vi "Autobuild Main.vi"() -> ()   [LabVIEW 2022 SP3]
uses:
  subVIs/Package Builder API/build type.ctl
  subVIs/Package Builder API/NI Package Builder API.lvlib
panel:
  out "current build":i32
  out "total builds":i32
  in  "Build Package":bool=TRUE
  in  "Build EXEs":bool=TRUE
  in  "Tab Control":T1(tab)
  in  "Projects":path[](array[path])=[path "C:/dev/class-d-amplifier/source/crosstalk/Crosstalk_Class D Amplifier.lvproj", path "C:/dev/class-d-amplifier/source/single tone/Single Tone Measurements_Class D Amplifier.lvproj", path "C:/dev/class-d-amplifier/source/stepped frequency sweep/Stepped Frequency Sweep_Class D Amplifier.lvproj", path "C:/dev/class-d-amplifier/source/efficiency/Efficiency_Class D Amplifier.lvproj", path "C:/dev/class-d-amplifier/source/efficiency sweep/Efficiency Sweep_Class D Amplifier.lvproj", path "C:/dev/class-d-amplifier/source/generation/Generation_Class D Amplifier.lvproj", path "C:/dev/class-d-amplifier/source/single tone no gen/Single Tone No Gen_Class D Amplifier.lvproj", path "C:/dev/class-d-amplifier/source/single tone power sweep/Single Tone Power Sweep.lvproj", path "C:/dev/class-d-amplifier/source/noise sweep/Noise Sweep_Class D Amplifier.lvproj", path "C:/dev/class-d-amplifier/source/crosstalk sweep/Crosstalk Sweep.lvproj"]
  in  "background service":path=path "C:/dev/class-d-amplifier/source/service/generation/Audio Generation Service.lvproj"
  in  "utilities":path=path "C:/dev/class-d-amplifier/source/service/register service/RegisterServices.lvproj"
  out "command line standard output":string
  in  "package builder solution path":path=path "C:/dev/class-d-amplifier/package/ClassDAmplifier.pbs"
  in  "error in (no error)":errorcluster
  out "error out":errorcluster
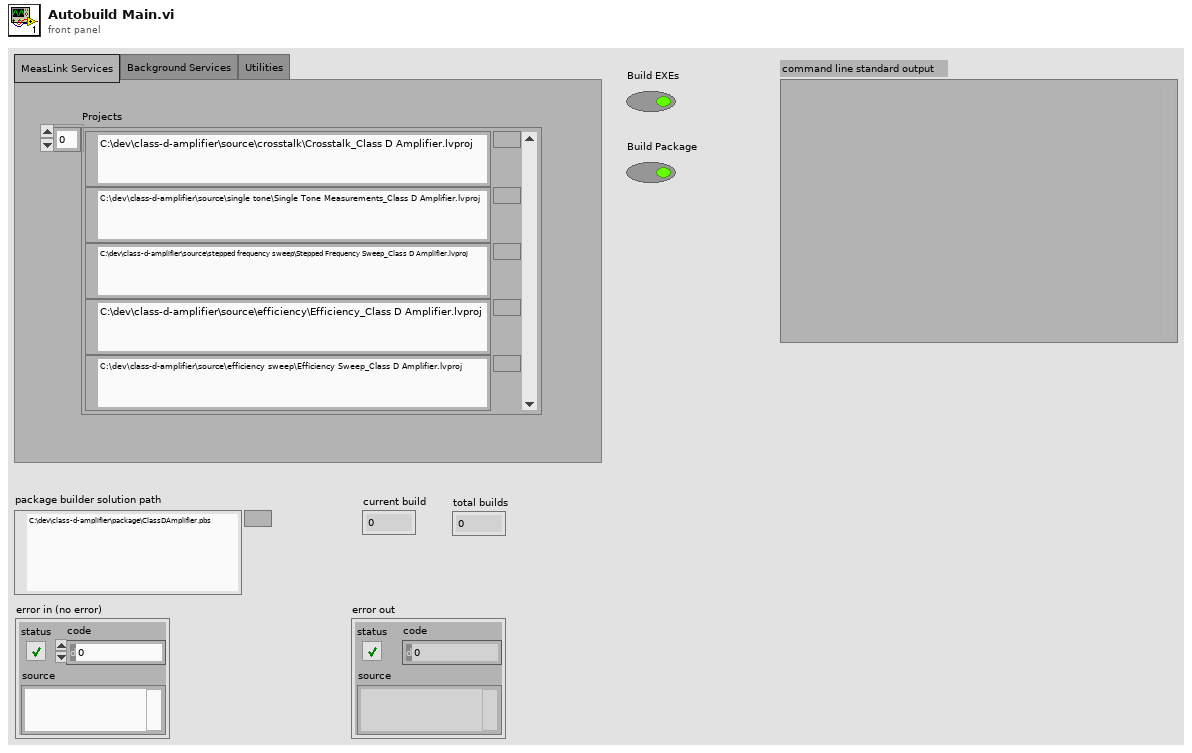
[diagram p1: front panel]
types:
  T1 = enum32{"MeasLink Services", "Background Services", "Utilities"}
  T2 = typedef "NI Package Builder API.lvlib/build type.ctl" = enum16{"packages", "feeds", "solution"}
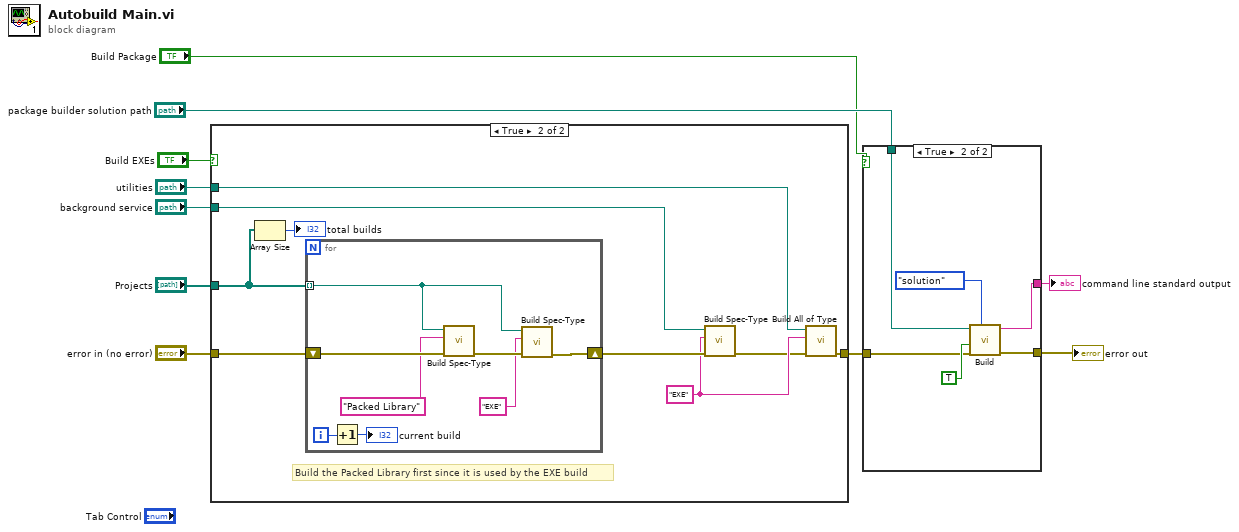
[diagram p0: block diagram]
diagram:
  n1 = case shown="True" "Build EXEs" {
    tunnel: "background service" -> [_ w19]
    tunnel: "utilities" -> [_ w16]
    tunnel: [w11 w15] -> w5
    tunnel: "error in (no error)" -> [w11 w14]
    tunnel: "Projects" -> [_ w13]
    frame False {
    }
    frame True {
      w18 = "EXE" ("Type")
      # "Build the Packed Library first since it is used by the EXE build"
      n2 = Array Size(array=w13) -> (size(s)=→"total builds":i32)
      n3 = for {
        shift-right: [w24] -> w20
        shift-left: w14 -> [w28]
        tunnel: w13 -> [w23] mode=indexing
        i -> [w22]
        n4 = Increment(x=w22) -> (x+1=→"current build":i32)
        n5 = call "Build Spec-Type.vi"("error in (no error)"=w28, "Type"="Packed Library", "Path to project"=w23) -> ("error out"=w27:errorcluster)  [unwired: 8 in]
        n6 = call "Build Spec-Type.vi"("error in (no error)"=w27, "Type"="EXE", "Path to project"=w23) -> ("error out"=w24:errorcluster)  [unwired: 8 in]
      }
      n7 = call "Build Spec-Type.vi"("error in (no error)"=w20, "Type"=w18, "Path to project"=w19) -> ("error out"=w17:errorcluster)  [unwired: 8 in]
      n8 = call "Build All of Type.vi"("error in (no error)"=w17, "Type"=w18, "Path to project"=w16) -> ("error out"=w15:errorcluster)  [unwired: 8 in]
    }
  }
  n9 = case shown="True" "Build Package" {
    tunnel: [w29 w35] -> w10
    tunnel: "package builder solution path" -> [_ w34]
    tunnel: [_ w33] -> w8
    tunnel: w5 -> [w29 w30]
    frame False {
    }
    frame True {
      n10 = call "Build.vi"("bulid type"=build_type."solution", "error in (no error)"=w30, "save build info to solution"=TRUE, "package builder solution path"=w34) -> ("error out"=w35:errorcluster, "command line standard output"=w33:string)  [unwired: 6 in]
    }
  }
  "error out" <- w10
  "command line standard output" <- w8
